vi "Example Grey.vi"() -> ()   [LabVIEW 2020]
uses:
  <vilib>/Utility/sysdir.llb/System Directory Type.ctl
  Sources/_Helpers/Tiff Page Details.ctl
  Sources/_Helpers/Tiff Data Type.ctl
  <vilib>/Analysis/Matrix/Datatypes/RealMatrix.ctl
  <vilib>/Analysis/1siggen.llb/Ramp Pattern by Samples.vi
  Sources/TIFF Writer/TIFF Writer.lvclass
  Sources/LV Tiff.lvlib
  Sources/TIFF Reader/TIFF Reader.lvclass
  <vilib>/Analysis/NI_AALBase.lvlib
  <vilib>/Analysis/Matrix/NI_Matrix.lvlib
panel:
  out "output array":dbl[][](array[numeric])
  out "DBL":dbl[][](graph)
  out "Read DBL":dbl[][](graph)
  out "U8":u8[][](graph)
  out "Read U8":u8[][](graph)
  out "Read U16":u16[][](graph)
  out "U16":u16[][](graph)
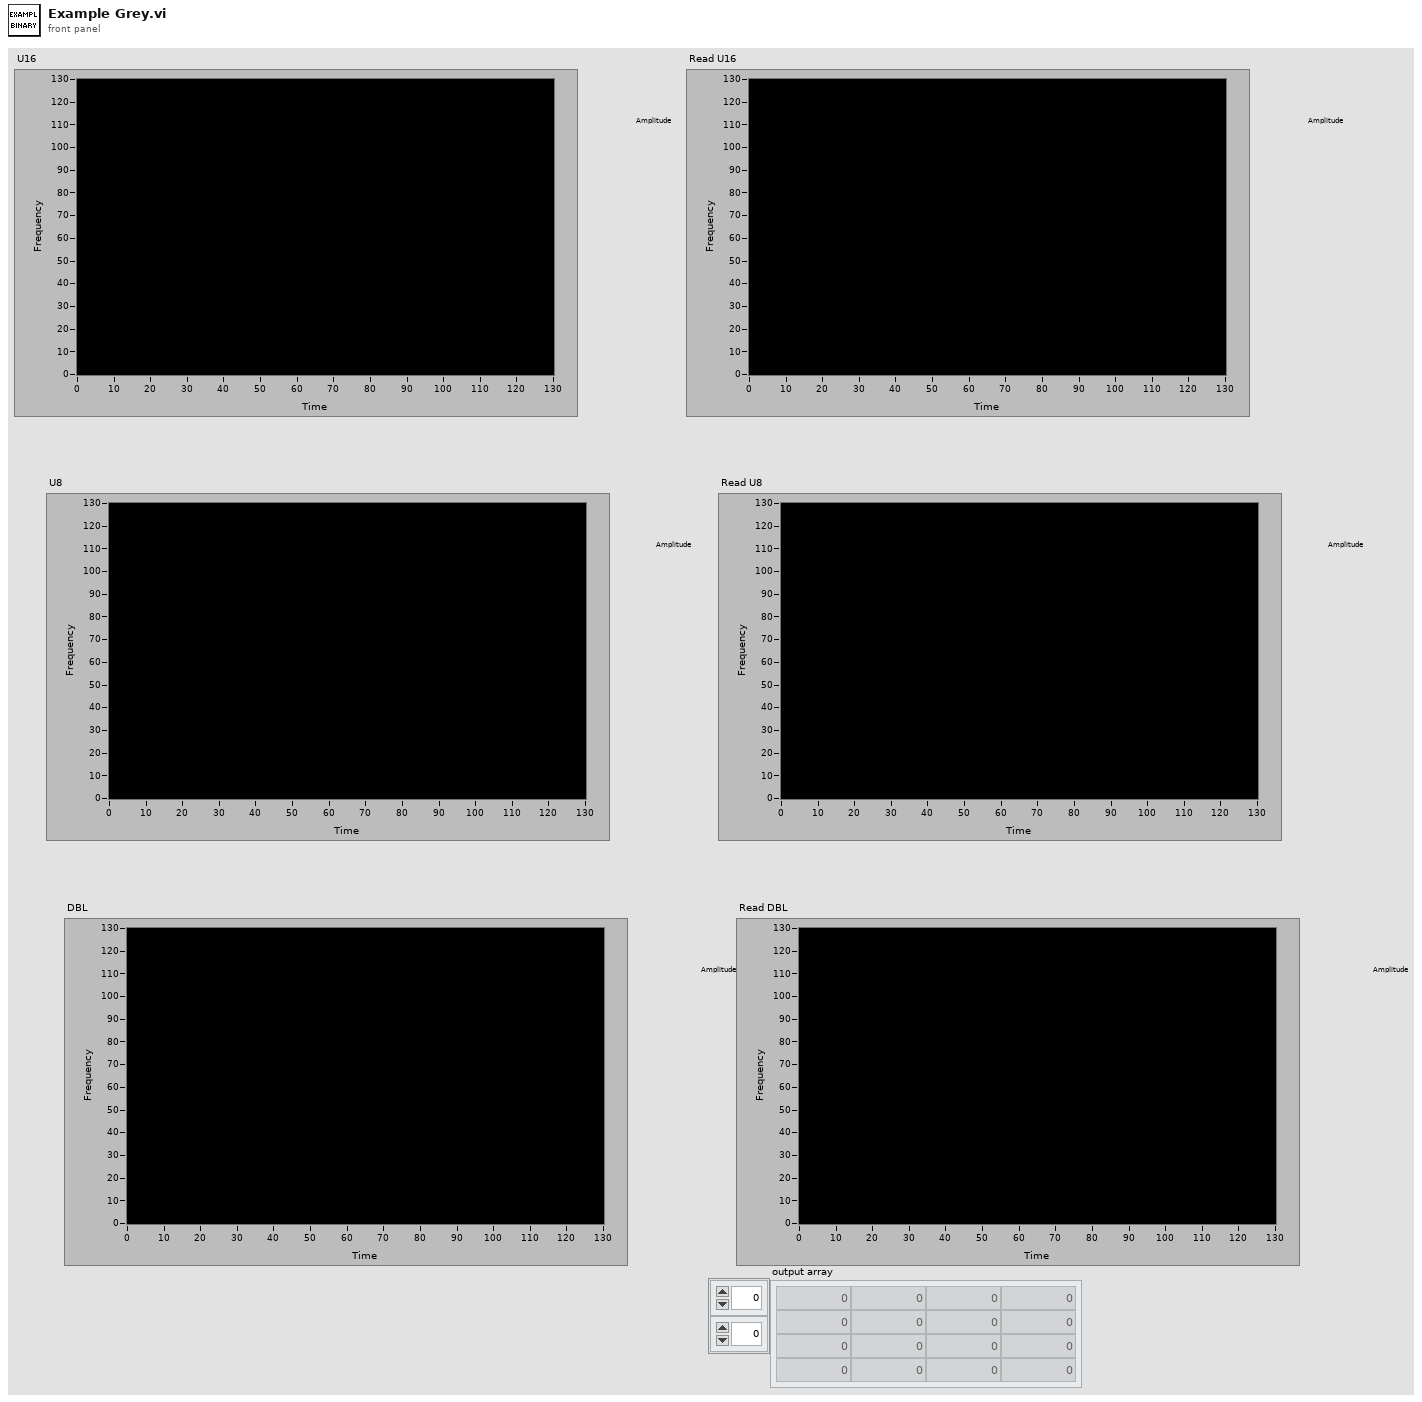
[diagram p1: front panel]
types:
  T1 = typedef "LV Tiff.lvlib/Tiff Data Type.ctl" = enum16{"Null", "BYTE", "ASCII", "SHORT", "LONG", "RATIONAL", "SBYTE", "UNDEFINE", "SSHORT", "SLONG", "SRATIONAL", "FLOAT", "DOUBLE"}
  T2 = typedef "NI_Matrix.lvlib/RealMatrix.ctl" = dbl[][]
  T3 = cluster{"Tag ID":i32, "Variant":variant, "DataType":T1}
  T4 = typedef "LV Tiff.lvlib/Tiff Page Details.ctl" = cluster{"ImageDescription":string, "XResolution":dbl, "YResolution":dbl, "ResolutionUnit":enum16{"None", "Inch", "Centimeter"}, "PhotometricInterpretation":u16, "Compression":enum16{"None", "Deflate", "JPEG"}, "PageName":string, "DocumentName":string}
  T5 = enum16{"open", "replace", "create", "open or create", "replace or create", "replace or create with confirmation"}
  T6 = typedef "System Directory Type.ctl" = i32
  T7 = cluster{"Tag ID":i32, "Variant":variant, "DataType":T1}[]
  T8 = cluster{cluster{"Tag ID":i32, "Variant":variant, "DataType":T1}[]}[]
  T9 = map{u16, cluster{"DataType":T1, "DataCount":u32, "DataOffset":u32}}
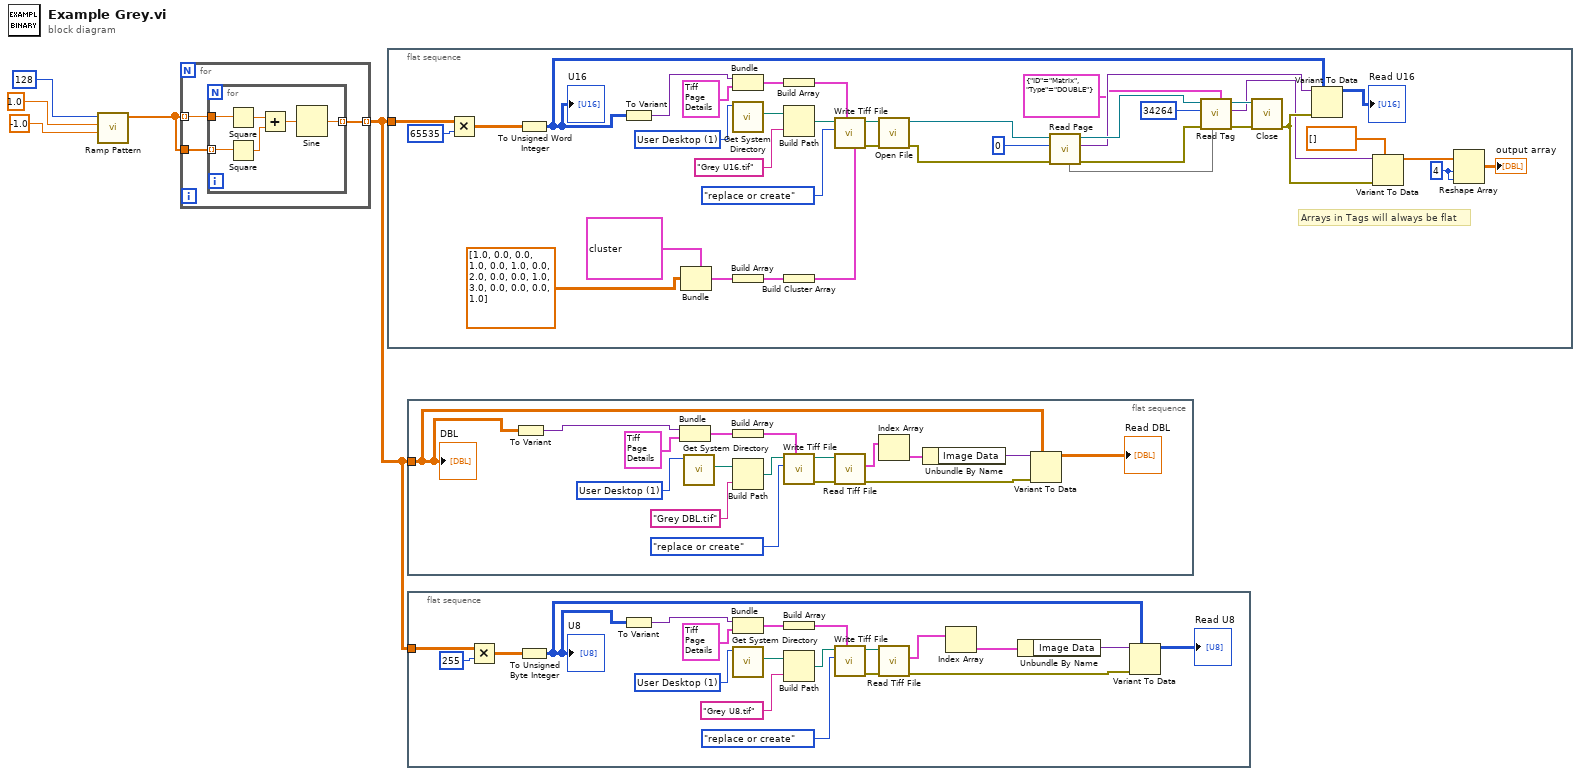
[diagram p0: block diagram]
diagram:
  n1 = call-poly <vilib>:"Ramp Pattern.vi"("start"=-1.0, "end"=1.0, "samples"=128) -> ("Ramp Pattern"=w2:dbl[])  [unwired: 7 in, 1 out]
  n2 = for {
    tunnel: [w8] -> w1 mode=indexing
    tunnel: w2 -> [w7] mode=indexing
    tunnel: w2 -> [w6]
    n3 = for {
      tunnel: [w14] -> w8 mode=indexing
      tunnel: w7 -> [w11]
      tunnel: w6 -> [w10] mode=indexing
      n4 = Square(x=w11) -> (x^2=w12:dbl)
      n5 = Square(x=w10) -> (x^2=w13:dbl)
      n6 = Add(x=w12, y=w13) -> (x+y=w9:dbl)
      n7 = Sine(x=w9) -> (sin(x)=w14:dbl)
    }
  }
  n8 = flat-sequence {
    tunnel: w1 -> [w43]
    frame #0 {
      w17 = 4 ("dimension size")
      w40 = T6 1 items=["User Home"=0, "User Desktop"=1, "User Documents"=2, "User Application Data"=3, "User Preferences"=4, "User Temporary"=5, "Public Documents"=6, "Public Application Data"=7, "Public Preferences"=8, "Public Cache"=13, "System Core Libraries"=9, "System Installed Libraries"=10, "Application Files"=11, "Boot Volume Root"=12] ("system directory type")
      # "Arrays in Tags will always be flat"
      n9 = Multiply(x=w43, y=u16 65535) -> (x*y=w51:dbl[][])
      n10 = To Unsigned Word Integer(number=w51) -> (unsigned 16bit integer=w52:u16[][])
      "U16" <- w52
      n11 = To Variant(anything=w52) -> (Variant=w47:variant)
      n12 = Bundle(cluster=T3 {"Tag ID"=34264, "Variant"=variant, "DataType"=enum."DOUBLE"}, "Variant"=T2 [[1.0, 0.0, 0.0, 1.0], [0.0, 1.0, 0.0, 2.0], [0.0, 0.0, 1.0, 3.0], [0.0, 0.0, 0.0, 1.0]] ("Input Matrix")) -> (w37:T3)  [unwired: 2 in]
      n13 = Bundle("Variant"=w47, "Details"=T4 {"ImageDescription"="", "XResolution"=0.0, "YResolution"=0.0, "ResolutionUnit"=enum."Inch", "PhotometricInterpretation"=34892, "Compression"=enum."None", "PageName"="", "DocumentName"=""}) -> (w48:cluster{"Variant":variant, "Details":T4})  [unwired: 1 in]
      n14 = call <vilib>:"Get System Directory.vi"("system directory type"=w40) -> ("system directory"=w45:path)  [unwired: 10 in]
      n15 = Build Array(w37) -> (w36:T7)
      n16 = Build Array(w48) -> (w49:cluster{"Variant":variant, "Details":T4}[])
      n17 = Build Path(base path=w45, name or relative path="Grey U16.tif") -> (appended path=w46:path)
      n18 = Build Cluster Array(w36) -> (w35:T8)
      n19 = call "Write Tiff File.vi"("Tags"=w35, "Pages"=w49, "operation (replace)"=T5."replace or create", "Path"=w46) -> ("error out"=w29:errorcluster, "path"=w31:path)  [unwired: 6 in]
      n20 = call "Open File.vi"("error in (no error)"=w29, "Path"=w31) -> ("error out"=w28:errorcluster, "TIFF Reader.lvclass"=w32:refnum<class "TIFF Reader.lvclass">)  [unwired: 7 in, 1 out]
      n21 = call "Read Page.vi"("error in (no error)"=w28, "index"=0, "TIFF Reader in"=w32) -> ("error out"=w27:errorcluster, "Image Data"=w30:variant, "TIFF Reader out"=w33:refnum<class "TIFF Reader.lvclass">, "IFD Info"=w24:T9)  [unwired: 4 in, 1 out]
      n22 = call "Read Tag.vi"("Override type"=cluster{"ID":string, "Type":T1} {"ID"="Matrix", "Type"=enum."DOUBLE"}, "IFD Info"=w24, "error in (no error)"=w27, "Tag ID"=34264 ("index"), "TIFF Reader in"=w33) -> ("error out"=w26:errorcluster, "Tag Data"=w20:variant, "TIFF Reader out"=w34:refnum<class "TIFF Reader.lvclass">)  [unwired: 3 in, 1 out]
      n23 = call "Close.vi"("error in (no error)"=w26, "TIFF Reader in"=w34) -> ("error out"=w21:errorcluster)  [unwired: 8 in, 1 out]
      n24 = Variant To Data(error in=w21, type=w52, Variant=w30) -> (data=→"Read U16":u16[][])  [unwired: 1 out]
      n25 = Variant To Data(error in=w21, type=dbl[] [] ("output array"), Variant=w20) -> (data=w18:dbl[])  [unwired: 1 out]
      n26 = Reshape Array(w18, w17, w17) -> (→"output array":dbl[][])
    }
  }
  n27 = flat-sequence {
    tunnel: w1 -> [w54]
    frame #0 {
      w56 = T6 1 items=["User Home"=0, "User Desktop"=1, "User Documents"=2, "User Application Data"=3, "User Preferences"=4, "User Temporary"=5, "Public Documents"=6, "Public Application Data"=7, "Public Preferences"=8, "Public Cache"=13, "System Core Libraries"=9, "System Installed Libraries"=10, "Application Files"=11, "Boot Volume Root"=12] ("system directory type")
      n28 = To Variant(anything=w54) -> (Variant=w61:variant)
      n29 = Bundle("Variant"=w61, "Details"=T4 {"ImageDescription"="", "XResolution"=0.0, "YResolution"=0.0, "ResolutionUnit"=enum."Inch", "PhotometricInterpretation"=34892, "Compression"=enum."None", "PageName"="", "DocumentName"=""}) -> (w62:cluster{"Variant":variant, "Details":T4})  [unwired: 1 in]
      n30 = call <vilib>:"Get System Directory.vi"("system directory type"=w56) -> ("system directory"=w59:path)  [unwired: 10 in]
      n31 = Build Array(w62) -> (w63:cluster{"Variant":variant, "Details":T4}[])
      n32 = Build Path(base path=w59, name or relative path="Grey DBL.tif") -> (appended path=w60:path)
      n33 = call "Write Tiff File.vi"("Pages"=w63, "operation (replace)"=T5."replace or create", "Path"=w60) -> ("error out"=w65:errorcluster, "path"=w64:path)  [unwired: 7 in]
      n34 = call "Read Tiff File.vi"("error in (no error)"=w65, "Path"=w64) -> ("error out"=w53:errorcluster, "Pages"=w66:cluster{"Image Data":variant, "Details":T4}[])  [unwired: 6 in, 2 out]
      n35 = Index Array(array=w66) -> (element=w67:cluster{"Image Data":variant, "Details":T4})  [unwired: 1 in]
      n36 = Unbundle By Name(w67) -> ("Image Data"=w68:variant)
      n37 = Variant To Data(error in=w53, type=w54, Variant=w68) -> (data=→"Read DBL":dbl[][])  [unwired: 1 out]
      "DBL" <- w54
    }
  }
  n38 = flat-sequence {
    tunnel: w1 -> [w75]
    frame #0 {
      w72 = T6 1 items=["User Home"=0, "User Desktop"=1, "User Documents"=2, "User Application Data"=3, "User Preferences"=4, "User Temporary"=5, "Public Documents"=6, "Public Application Data"=7, "Public Preferences"=8, "Public Cache"=13, "System Core Libraries"=9, "System Installed Libraries"=10, "Application Files"=11, "Boot Volume Root"=12] ("system directory type")
      n39 = Multiply(x=w75, y=u8 255) -> (x*y=w88:dbl[][])
      n40 = To Unsigned Byte Integer(number=w88) -> (unsigned 8bit integer=w89:u8[][])
      "U8" <- w89
      n41 = To Variant(anything=w89) -> (Variant=w79:variant)
      n42 = Bundle("Variant"=w79, "Details"=T4 {"ImageDescription"="", "XResolution"=0.0, "YResolution"=0.0, "ResolutionUnit"=enum."Inch", "PhotometricInterpretation"=34892, "Compression"=enum."None", "PageName"="", "DocumentName"=""}) -> (w80:cluster{"Variant":variant, "Details":T4})  [unwired: 1 in]
      n43 = call <vilib>:"Get System Directory.vi"("system directory type"=w72) -> ("system directory"=w77:path)  [unwired: 10 in]
      n44 = Build Array(w80) -> (w81:cluster{"Variant":variant, "Details":T4}[])
      n45 = Build Path(base path=w77, name or relative path="Grey U8.tif") -> (appended path=w78:path)
      n46 = call "Write Tiff File.vi"("Pages"=w81, "operation (replace)"=T5."replace or create", "Path"=w78) -> ("error out"=w83:errorcluster, "path"=w82:path)  [unwired: 7 in]
      n47 = call "Read Tiff File.vi"("error in (no error)"=w83, "Path"=w82) -> ("error out"=w70:errorcluster, "Pages"=w84:cluster{"Image Data":variant, "Details":T4}[])  [unwired: 6 in, 2 out]
      n48 = Index Array(array=w84) -> (element=w85:cluster{"Image Data":variant, "Details":T4})  [unwired: 1 in]
      n49 = Unbundle By Name(w85) -> ("Image Data"=w86:variant)
      n50 = Variant To Data(error in=w70, type=w89, Variant=w86) -> (data=→"Read U8":u8[][])  [unwired: 1 out]
    }
  }
